vi "JKI State Machine Helper.vi"(6 "Variant in":variant, 7 "Shift Pressed?":bool, 8 "error in (no error)":errorcluster, 10 "QD Combo Box Ref":refnum<vi>, 11 "QD Launch VI Ref":refnum<vi>) -> (0 "error out":errorcluster, 4 "Variant out":variant)   [LabVIEW 2020]
doc: "Launches JKI State Machine Helper.\n\nDefault Shortcut - [j]"
uses:
  JKI State Machine API/source/JKI SM/JKI SM.lvclass
panel:
  in  "Undo Name":string="Quick Drop Keyboard Shortcut"
  # "Do not change the connector pane of this VI.\n\nSee the block diagram for directions on how to use this template."
  # "Specify the name of the Undo transaction"
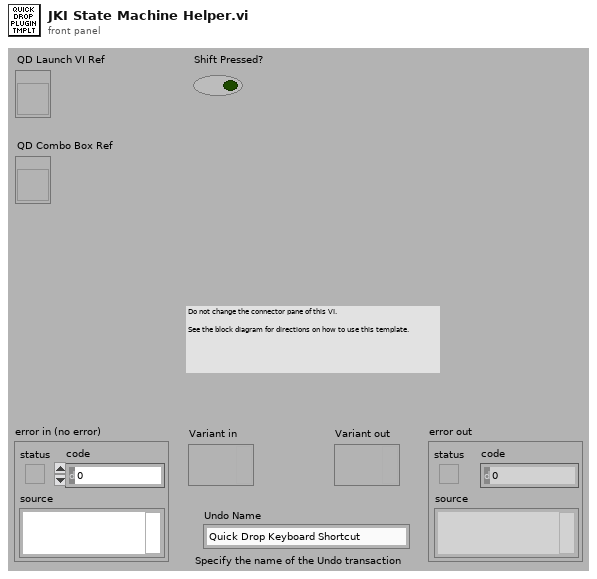
[diagram p1: front panel]
types:
  T1 = cluster{"App.ContextName":string, "VI.Name":string, "Object UID":i32}
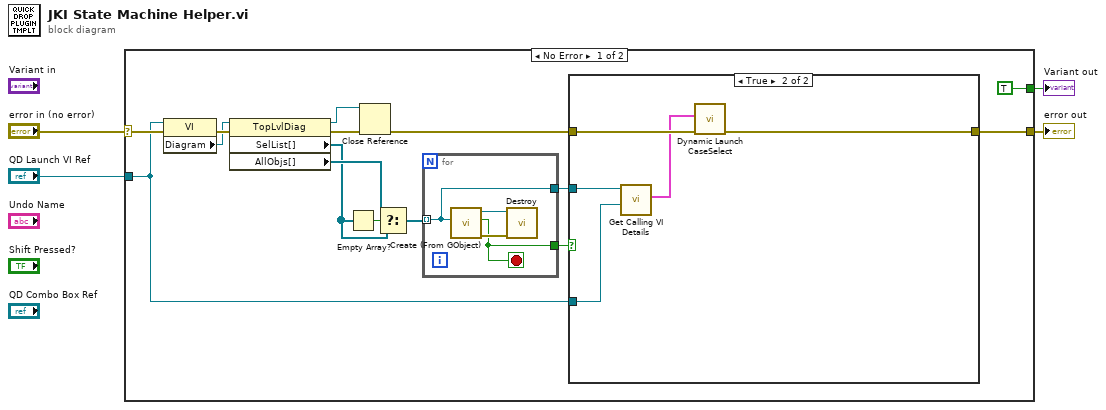
[diagram p0: block diagram]
diagram:
  n1 = case shown="No Error" "error in (no error)" {
    selector: "error in (no error)" -> [w19 w30]
    tunnel: [w12 w30] -> w3
    tunnel: "QD Launch VI Ref" -> [w5 _]
    tunnel: [TRUE _] -> w1
    frame No Error {
      n2 = property class="VI"(reference=w5, error in=w19) -> (error out=w16:errorcluster, "Diagram"=w15:refnum<vi>)  [unwired: 1 out]
      n3 = property class="TopLvlDiag"(reference=w15, error in=w16) -> (reference out=w13:refnum<vi>, error out=w14:errorcluster, "SelList[]"=w8:refnum<vi>[], "AllObjs[]"=w10:refnum<vi>[])
      n4 = Empty Array?(array=w8) -> (empty?=w11:bool)
      n5 = Close Reference(reference=w13, error in (no error)=w14) -> (error out=w17:errorcluster)
      n6 = Select(t=w10, s=w11, f=w8) -> (s? t:f=w9:refnum<vi>[])
      n7 = for {
        tunnel: w9 -> [w27] mode=indexing
        tunnel: [w27] -> w6
        tunnel: [w26] -> w7
        stop <- w26 stop-if-true
        n8 = call "Create (From GObject).vi"("GObject"=w27) -> ("error out"=w28:errorcluster, "Found JKI SMs?"=w26:bool, "JKI SM out"=w29:refnum<class "JKI SM.lvclass">)  [unwired: 7 in, 1 out]
        n9 = call "Destroy.vi"("error in (no error)"=w28, "JKI SM in"=w29) -> ()  [unwired: 9 in, 1 out]
      }
      n10 = case shown="True" w7 {
        tunnel: w17 -> [w20 w25]
        tunnel: [w20 w24] -> w12
        tunnel: w6 -> [_ w23]
        tunnel: w5 -> [_ w22]
        frame False {
        }
        frame True {
          n11 = call "Get Calling VI Details.vi"("User VI Ref"=w22, "Affected Items"=w23) -> ("Calling VI Details"=w21:T1)  [unwired: 9 in]
          n12 = call "Dynamic Launch CaseSelect.vi"("error in (no error)"=w25, "Owning VI Details"=w21) -> ("error out"=w24:errorcluster)  [unwired: 9 in]
        }
      }
    }
    frame Error {
    }
  }
  "error out" <- w3
  "Variant out" <- w1
